vi "PicoScope5000aExampleBlockMSO.vi"() -> ()   [LabVIEW 2010]
uses:
  shared/PicoBuffers.ctl
  <vilib>/Waveform/DWDTOps.llb/DWDT Analog to Digital.vi
  PicoScope5000aLib/PicoScope5000aAnalogChannelSettings.ctl
  shared/Buffer and Transfer Settings.ctl
  shared/Acquisition Settings.ctl
  PicoScope5000aLib/PicoScope5000aDigitalChannelSettings.ctl
panel:
  out "overflow":i16 format="%010b"
  in  "Apply Settings":bool
  in  "Port 0 Settings":T1={"Enabled"=FALSE, "Logic Level"=9830} {"Logic Level" items=["1.5V TTL"=9830, "2.5V CMOS"=16383]}
  in  "Channel A Settings":T2={"Enabled"=TRUE, "Coupling"=1, "Range"=6, "Analogue Offset"=0.0, "Bandwidth Limit"=0} {"Bandwidth Limit" items=["Full", "20MHz"]; "Range" items=["10 mV", "20 mV", "50 mV", "100 mV", "200 mV", "500 mV", "1 V", "2 V", "5 V", "10 V", "20 V"]; "Coupling" items=["AC", "DC"]}
  in  "Trigger Settings":T3={"Trigger Enabled"=FALSE, "Trigger Source"=enum."Channel A", "Trigger Threshold (volts)"=0.0, "Trigger Direction"=2, "Trigger Delay (samples)"=0, "Auto Trigger Time (ms)"=1000} {"Trigger Direction" items=["Rising"=2, "Falling"=3]}
  out "USB 3.0 device on non-USB 3.0 Port":bool=TRUE
  out "USB Powered":bool=TRUE
  out "Device Info":T4={"Driver Version"="2.1.104.3324", "USB Version"="2.0", "Hardware"="1", "Variant"="5244A", "Batch and Serial"="CQ178/007", "Cal Date"="11Jun13", "Kernel Version"="1.0", "Digital HW Version"="1", "Analogue HW Version"="1", "MSO"=FALSE, "Number of channels"=2}
  out "error out":errorcluster
  in  "Data file":path=path "PicoScope5000aExampleBlock ChA Data"
  in  "Buffer and Transfer Settings":T5={"startIndex"=0, "Samples"=5000000, "Down Sample Ratio"=1, "Down-Sample Mode"=0} {"Down-Sample Mode" items=["RAW none"=2147483648, "None"=0, "Aggregate"=1, "Decimate"=2, "Average"=4]; "Down Sample Ratio" step=1; "Samples" format="%_6p"}
  in  "Acquisition Settings":T6={"preTriggerSamples"=0, "postTriggerSamples"=5000000, "timebase"=5} {"postTriggerSamples" format="%_6p"; "preTriggerSamples" format="%_6p"}
  out "Properties Panel":T7={"Sample Frequency"=41666668.0, "Sample Rate"=2.4000000209412065e-08, "Max Samples Available"=26843008, "Number of Samples"=0, "Total Capture Time (sec) "=0.0, "Max Total Capture Time Available (sec)"=0.6442322134971619} {"Max Total Capture Time Available (sec)" format="%.3p"; "Sample Frequency" format="%.6p"; "Sample Rate" format="%.3p"; "Max Samples Available" format="%_6p"; "Total Capture Time (sec)" format="%.3p"}
  out "Port 0":digitalwaveform(graph)={"t0"=timestamp(0 s since 1904-01-01), "dt"=8e-09, "Y"={"transitions"=[], "data"=[]}}
  in  "stop":bool
  out "Analog Channels":cluster{i32, sgl, "Data":dbl[]}[](graph)
  in  "Resolution":u32(ring) items=["8-bit"=0, "12-bit"=1, "14-bit"=2, "15-bit"=3, "16-bit"=4, "10-bit"=10]
  in  "Serial Number":string
  in  "Use Serial Number":bool
  in  "error in (no error)":errorcluster
  # "Bit 0 = ChA"
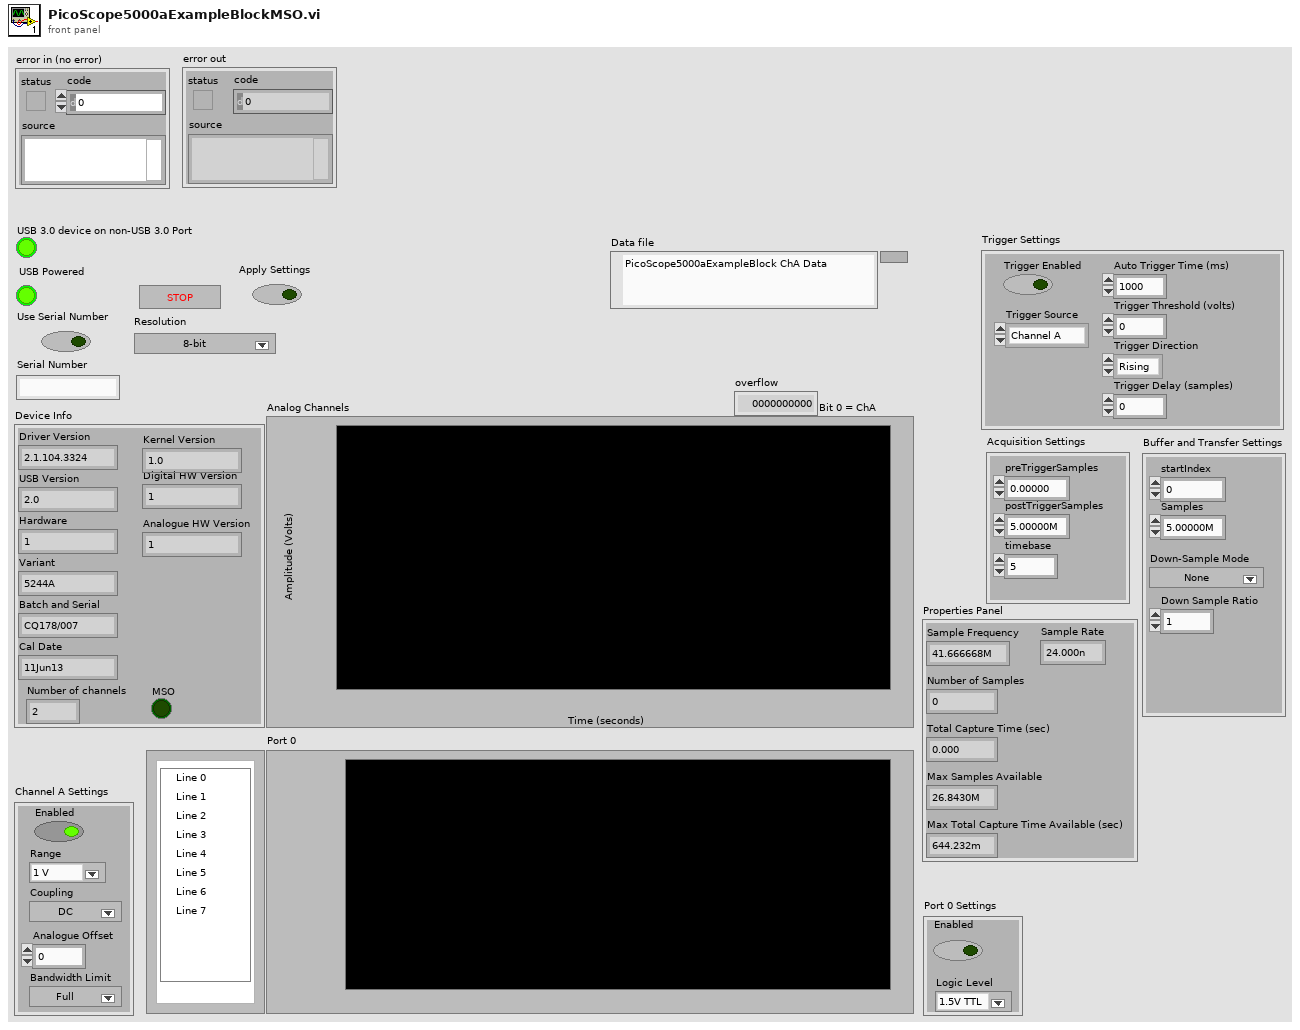
[diagram p1: front panel]
types:
  T1 = typedef "PicoScope5000aDigitalChannelSettings.ctl" = cluster{"Enabled":bool, "Logic Level":i16}
  T2 = typedef "PicoScope5000aAnalogChannelSettings.ctl" = cluster{"Enabled":bool, "Coupling":i16, "Range":u16, "Analogue Offset":sgl, "Bandwidth Limit":u32}
  T3 = cluster{"Trigger Enabled":bool, "Trigger Source":enum16{"Channel A", "Channel B", "Channel C", "Channel D", "Ext."}, "Trigger Threshold (volts)":dbl, "Trigger Direction":u16, "Trigger Delay (samples)":u32, "Auto Trigger Time (ms)":i16}
  T4 = cluster{"Driver Version":string, "USB Version":string, "Hardware":string, "Variant":string, "Batch and Serial":string, "Cal Date":string, "Kernel Version":string, "Digital HW Version":string, "Analogue HW Version":string, "MSO":bool, "Number of channels":i16}
  T5 = typedef "Buffer and Transfer Settings.ctl" = cluster{"startIndex":u64, "Samples":u64, "Down Sample Ratio":u64, "Down-Sample Mode":u32}
  T6 = typedef "Acquisition Settings.ctl" = cluster{"preTriggerSamples":u64, "postTriggerSamples":u64, "timebase":u32}
  T7 = cluster{"Sample Frequency":dbl, "Sample Rate":dbl, "Max Samples Available":u64, "Number of Samples":u64, "Total Capture Time (sec) ":dbl, "Max Total Capture Time Available (sec)":dbl}
  T8 = enum16{"open", "open or create", "create or replace", "create", "open (read-only)"}
  T9 = typedef "PicoBuffers.ctl" = cluster{"Max Buffer Pointers":u64[][][], "Min Buffer Pointers":u64[][][], "StreamingDataInfo":cluster{"Channel":u32, "Down-Sample Mode":u32, "PICO_DATA_TYPE":enum32{"PICO_INT8_T", "PICO_INT16_T", "PICO_INT32_T", "PICO_UINT32_T", "PICO_INT64_T", ""}, "Samples":i32, "bufferIndex":u64, "startIndex":i32, "overflow":i16}[][]}
  T10 = cluster{"Sample Frequency":sgl, "Sample Rate":sgl, "Max Samples Available":i32, "Number of Samples":u32, "Total Capture Time (sec) ":sgl, "Max Total Capture Time Available (sec)":sgl}
  T11 = cluster{"Channel A Buffer":i16[], "Channel B Buffer":i16[], "Channel C Buffer":i16[], "Channel D Buffer":i16[], "Channel E Buffer":i16[], "Channel F Buffer":i16[], "Channel G Buffer":i16[], "Channel H Buffer":i16[], "Port 0 Buffer":i16[], "Port 1 Buffer":i16[]}[]
  T12 = cluster{"Channel A Buffer":i16[], "Channel B Buffer":i16[], "Channel C Buffer":i16[], "Channel D Buffer":i16[], "Channel E Buffer":i16[], "Channel F Buffer":i16[], "Channel G Buffer":i16[], "Channel H Buffer":i16[], "Port 0 Buffer":i16[], "Port 1 Buffer":i16[]}
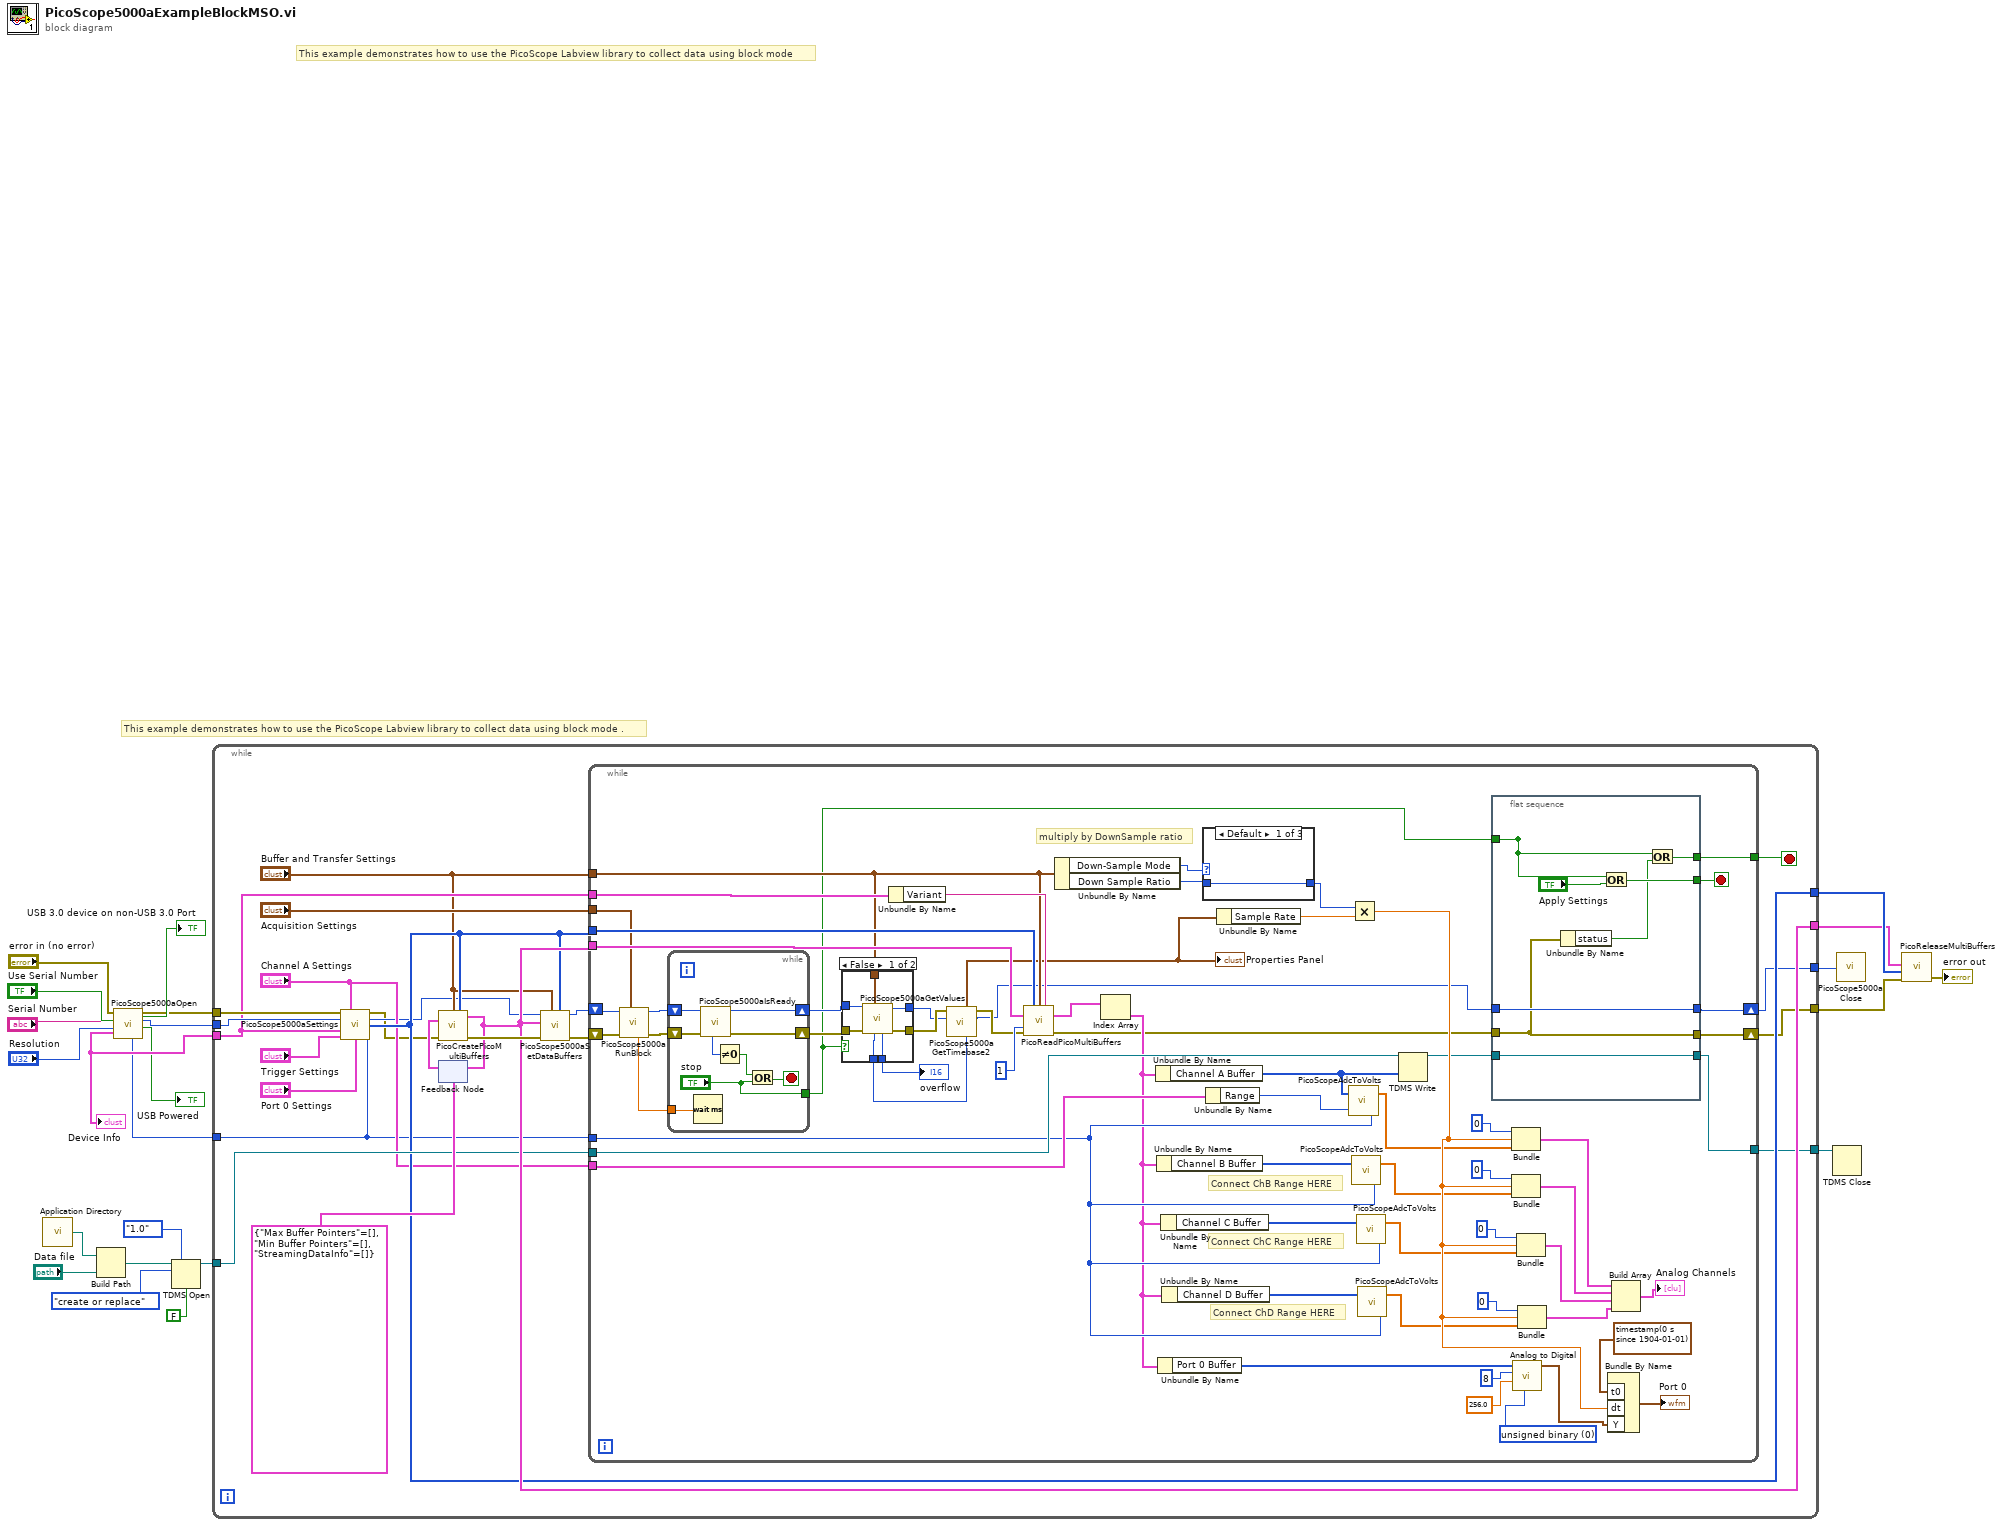
[diagram p0: block diagram]
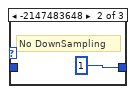
[diagram p3: hidden frame]
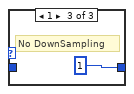
[diagram p4: hidden frame]
diagram:
  # "This example demonstrates how to use the PicoScope Labview library to collect data using block mode ."
  # "This example demonstrates how to use the PicoScope Labview library to collect data using block mode"
  n1 = call <vilib>:"Application Directory.vi"() -> ("Application Directory"=w15:path)
  n2 = Build Path(base path=w15, name or relative path="Data file") -> (appended path=w16:path)
  n3 = call "PicoScope5000aOpen.vi"("Serial Number"="Serial Number", "Resolution"="Resolution", "Use Serial Number"="Use Serial Number", "error in (no error)"="error in (no error)") -> ("USB Powered"=→"USB Powered":bool, "handle"=w23:i16, "error out"=w3:errorcluster, "Max ADC value"=w6:i16, "USB 3.0 device on non-USB 3.0 Port"=→"USB 3.0 device on non-USB 3.0 Port":bool, "Device Info"=w7:T4)  [unwired: 2 in]
  "Device Info" <- w7
  n4 = TDMS Open(6:FALSE ("disable buffering? (T)"), 7:enum16{"1.0", "2.0"}."1.0" ("file format version (2.0)"), 10:T8."create or replace" ("operation (0:open)"), 11:w16) -> (3:w13:refnum<k34>)  [unwired: 2 in, 1 out]
  n5 = while {
    tunnel: w23 -> [w41]
    tunnel: w6 -> [w34]
    tunnel: [w38] -> w22
    tunnel: [w43] -> w21
    tunnel: [w31] -> w14
    tunnel: w13 -> [w42]
    tunnel: w7 -> [w33]
    tunnel: w3 -> [w40]
    tunnel: [w32] -> w2
    tunnel: [w29] -> w1
    stop <- w30 stop-if-true
    n6 = call "PicoScope5000aSettings.vi"("error in"=w40, "Channel A Settings"="Channel A Settings", "Port 0 Settings"="Port 0 Settings", "handle in"=w41, "Device Info"=w33, "Trigger Settings"="Trigger Settings", "Max ADC value"=w34) -> ("error out"=w24:errorcluster, "handle out"=w25:i16, "enabled array"=w38:i16[])  [unwired: 6 in]
    n7 = feedback #1(T9 {"Max Buffer Pointers"=[], "Min Buffer Pointers"=[], "StreamingDataInfo"=[]} ("Data Pointers")) -> (w45:T9)
    n8 = call "PicoCreatePicoMultiBuffers.vi"("Buffer and Transfer Settings"="Buffer and Transfer Settings", "enabled array"=w38, "Data Pointers In"=w45, "error in (no error)"=w24) -> ("Data Pointers"=w43:T9, "error out"=w44:errorcluster)  [unwired: 10 in]
    n9 = feedback-in #1(w43) -> ()
    n10 = call "PicoScope5000aSetDataBuffers.vi"("enabled array"=w38, "Buffer and Transfer Settings"="Buffer and Transfer Settings", "error in (no error)"=w44, "Data Pointers In"=w43, "handle in"=w25) -> ("error out"=w28:errorcluster, "handle out"=w27:i16)  [unwired: 5 in]
    n11 = while {
      tunnel: w43 -> [w110]
      tunnel: "Buffer and Transfer Settings" -> [w55]
      tunnel: w38 -> [w101]
      tunnel: "Channel A Settings" -> [w100]
      tunnel: "Acquisition Settings" -> [w99]
      tunnel: w34 -> [w98]
      tunnel: w33 -> [w95]
      tunnel: [w62] -> w30
      shift-right: [w66] -> w32
      shift-left: w28 -> [w56]
      shift-right: [w60] -> w29
      shift-left: w27 -> [w57]
      tunnel: w42 -> [w109]
      tunnel: [w64] -> w31
      stop <- w61 stop-if-true
      w83 = u16 0 items=["unsigned binary", "offset binary", "2's complement"] ("data format (offset binary)")
      # "Connect ChB Range HERE"
      # "Connect ChD Range HERE"
      # "Connect ChC Range HERE"
      # "multiply by DownSample ratio"
      n12 = call "PicoScope5000aRunBlock.vi"("Acquisition Settings"=w99, "error in (no error)"=w56, "handle in"=w57) -> ("error out"=w103:errorcluster, "handle out"=w102:i16, "timeIndisposedMs"=w93:dbl)  [unwired: 5 in, 1 out]
      n13 = while {
        shift-right: [w135] -> w58
        shift-left: w103 -> [w136]
        shift-right: [w134] -> w59
        shift-left: w102 -> [w133]
        tunnel: ["stop"] -> w54
        tunnel: w93 -> [w128]
        stop <- w130 stop-if-true
        n14 = Wait (ms)(milliseconds to wait=w128) -> ()  [unwired: 1 out]
        n15 = call "PicoScope5000aIsReady.vi"("error in (no error)"=w136, "handle in"=w133) -> ("error out"=w135:errorcluster, "handle out"=w134:i16, "ready"=w132:i16)  [unwired: 7 in]
        n16 = Not Equal To 0?(x=w132) -> (x != 0?=w131:bool)
        n17 = Or(x=w131, y="stop") -> (x .or. y?=w130:bool)
      }
      n18 = case shown="False" w54 {
        tunnel: w58 -> [w117 w118]
        tunnel: w59 -> [w116 w119]
        tunnel: [w115 w119] -> w51
        tunnel: [w114 w118] -> w52
        tunnel: w55 -> [w113 _]
        tunnel: [w112 _] -> w53
        tunnel: [w111 _] -> w48
        frame False {
          n19 = call "PicoScope5000aGetValues.vi"("Buffer and Transfer Settings"=w113, "error in (no error)"=w117, "handle in"=w116) -> ("error out"=w114:errorcluster, "handle out"=w115:i16, "overflow"=w112:i16, "noOfSamples"=w111:u64)  [unwired: 5 in]
        }
        frame True {
        }
      }
      "overflow" <- w53
      n20 = Unbundle By Name(w95) -> ("Variant"=w96:string)
      n21 = call "PicoScope5000aGetTimebase2.vi"("Number of Samples"=w48, "handle in"=w51, "error in (no error)"=w52) -> ("handle out"=w49:i16, "error out"=w50:errorcluster, "Properties Panel"=w47:T10)  [unwired: 6 in]
      "Properties Panel" <- w47
      n22 = call "PicoReadPicoMultiBuffers.vi"("enabled array"=w101, "Buffer and Transfer Settings"=w55, "Variant"=w96, "Data Pointers"=w110, "No of Buffers"=1, "error in (no error)"=w50) -> ("MultiBuffers (Max or non-aggregated)"=w108:T11, "error out"=w63:errorcluster)  [unwired: 7 in, 1 out]
      n23 = Unbundle By Name(w55) -> ("Down-Sample Mode"=w106:u32, "Down Sample Ratio"=w107:u64)
      n24 = Index Array(array=w108) -> (element=w67:T12)  [unwired: 1 in]
      n25 = Unbundle By Name(w67) -> ("Channel A Buffer"=w76:i16[])
      n26 = Unbundle By Name(w67) -> ("Channel B Buffer"=w89:i16[])
      n27 = Unbundle By Name(w67) -> ("Port 0 Buffer"=w81:i16[])
      n28 = Unbundle By Name(w67) -> ("Channel C Buffer"=w74:i16[])
      n29 = Unbundle By Name(w67) -> ("Channel D Buffer"=w70:i16[])
      n30 = case shown="Default" w106 {
        tunnel: [w137 u64 1 ("Down Sample Ratio") u64 1 ("Down Sample Ratio")] -> w104
        tunnel: w107 -> [w137 _ _]
        frame Default {
        }
        frame -2147483648 {
          # "No DownSampling"
        }
        frame 1 {
          # "No DownSampling"
        }
      }
      n31 = Unbundle By Name(w100) -> ("Range"=w91:u16)
      n32 = Unbundle By Name(w47) -> ("Sample Rate"=w97:sgl)
      n33 = call "PicoScopeAdcToVolts.vi"("Max_adc"=w98, "Range Index"=w91, "Data"=w76) -> ("Data"=w77:dbl[])
      n34 = Multiply(x=w104, y=w97) -> (x*y=w105:sgl)
      n35 = call "PicoScopeAdcToVolts.vi"("Max_adc"=w98, "Data"=w89) -> ("Data"=w88:dbl[])  [unwired: 1 in]
      n36 = call "PicoScopeAdcToVolts.vi"("Max_adc"=w98, "Data"=w74) -> ("Data"=w73:dbl[])  [unwired: 1 in]
      n37 = call "PicoScopeAdcToVolts.vi"("Max_adc"=w98, "Data"=w70) -> ("Data"=w69:dbl[])  [unwired: 1 in]
      n38 = TDMS Write(0:w109, 9:w76) -> (4:w65:refnum<k34>)  [unwired: 4 in, 3 out]
      n39 = flat-sequence {
        tunnel: [w127] -> w61
        tunnel: [w120] -> _
        tunnel: [w124] -> w62
        tunnel: w49 -> [w123]
        tunnel: [w123] -> w60
        tunnel: w63 -> [w122]
        tunnel: [w122] -> w66
        tunnel: [w121] -> w64
        tunnel: w65 -> [w121]
        tunnel: w54 -> [w120]
        frame #0 {
          n40 = Unbundle By Name(w122) -> ("status"=w125:bool)
          n41 = Or(x=w120, y="Apply Settings") -> (x .or. y?=w127:bool)
          n42 = Or(x=w120, y=w125) -> (x .or. y?=w124:bool)
        }
      }
      n43 = Bundle(0, w105, "Data"=w77) -> (w87:cluster{i32, sgl, "Data":dbl[]})  [unwired: 1 in]
      n44 = Bundle(0, w105, "Data"=w88) -> (w86:cluster{i32, sgl, "Data":dbl[]})  [unwired: 1 in]
      n45 = call-poly <vilib>:"Analog to Digital.vi"("data format (offset binary)"=w83, "full-scale range (pk-pk)"=256.0, "resolution (16 bit)"=8, "analog waveform"=w81) -> ("digital waveform"=w78:digitalwaveform)  [unwired: 4 in, 3 out]
      n46 = Bundle(0, w105, "Data"=w73) -> (w72:cluster{i32, sgl, "Data":dbl[]})  [unwired: 1 in]
      n47 = Bundle(0, w105, "Data"=w69) -> (w68:cluster{i32, sgl, "Data":dbl[]})  [unwired: 1 in]
      n48 = Bundle By Name("t0"=timestamp(0 s since 1904-01-01), "dt"=w105, "Y"=w78) -> (→"Port 0":digitalwaveform)  [unwired: 1 in]
      n49 = Build Array(w87, w86, w72, w68) -> (→"Analog Channels":cluster{i32, sgl, "Data":dbl[]}[])
    }
  }
  n50 = TDMS Close(11:w14) -> ()  [unwired: 1 in, 2 out]
  n51 = call "PicoScope5000aClose.vi"("handle"=w1) -> ()
  n52 = call "PicoReleaseMultiBuffers.vi"("error in (no error)"=w2, "Enabled array"=w22, "Data Pointers"=w21) -> ("error out"=→"error out":errorcluster)  [unwired: 8 in]
